vi "PicoScope3000aGetMaxEtsValues.vi"(8 "error in (no error)":errorcluster, 11 "handle in":i16) -> (0 "error out":errorcluster, 1 "Max etsInterleave":i16, 2 "Max etsCycles":i16, 3 "handle out":i16)   [LabVIEW 2010]
doc: "Calls GetMaxEtsValues"
uses:
  ps3000a.dll
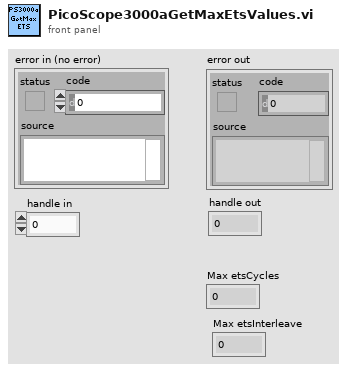
[diagram p1: front panel]
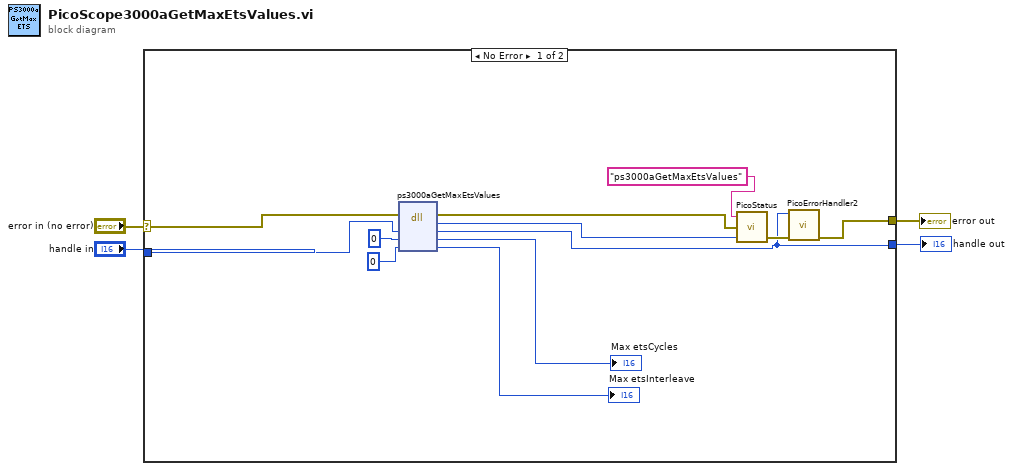
[diagram p0: block diagram]
diagram:
  n1 = case shown="No Error" "error in (no error)" {
    selector: "error in (no error)" -> [w9 w18]
    tunnel: [w15 w18] -> w2
    tunnel: "handle in" -> [w8 w17]
    tunnel: [w7 w17] -> w3
    frame No Error {
      n2 = dll-call lib="ps3000a.dll" fn="ps3000aGetMaxEtsValues" ("ps3000.dll:_ps3000_open_unit@0")(error in=w9, "handle"=w8, "etsCycles"=i16 0, "etsInterleave"=i16 0) -> (error out=w11:errorcluster, "PICO_STATUS"=w10:u32, "handle"=w7:i16, "etsCycles"=→"Max etsCycles":i16, "etsInterleave"=→"Max etsInterleave":i16)  [unwired: 2 in, 1 out]
      n3 = call "PicoStatus.vi"("PICO STATUS"=w10, "error in"=w11, "source"="ps3000aGetMaxEtsValues") -> ("error out"=w16:errorcluster)
      n4 = call "PicoErrorHandler2.vi"("error in (no error)"=w16, "handle In"=w7) -> ("error out"=w15:errorcluster)  [unwired: 9 in]
    }
    frame Error {
    }
  }
  "error out" <- w2
  "handle out" <- w3
